vi "Auto_PID_Drive.vi"(0 "Power":dbl, 1 "dt (s)":dbl=10.0 format="%.3f", 5 "Turning":dbl, 7 "PID Gains":T1={"P"=0.09, "I"=0.9, "D"=0.001, "F"=0.0, "IZone"=0.0}, 9 "Yaw":dbl=-13.119872265000097, 11 "Turning_Setpoint":dbl, 12 "Turning_PID_Enable":bool) -> (4 "Power":dbl, 6 "Turning":dbl)   [LabVIEW 2019, in "ArgosLib.lvlib"]
uses:
  ArgosLib.lvlib
  Config/ConfigComponents/TypeDefs/Config_PIDParams.ctl
  <vilib>/addons/control/pid/pid.llb/PID (DBL).vi
  <vilib>/Rock Robotics/Network Tables/NT Write Number.vi
  <vilib>/addons/control/pid/NI_PID_pid.lvlib
  <vilib>/Rock Robotics/Network Tables/NT Read Number.vi
panel:
  out "Error":dbl
  out "Waveform Chart 2":dbl(graph)
  out "Waveform Chart":cluster{"Turning_Setpoint":dbl, "Yaw":dbl}(graph)={"Turning_Setpoint"=0.0, "Yaw"=-13.119872265000097}
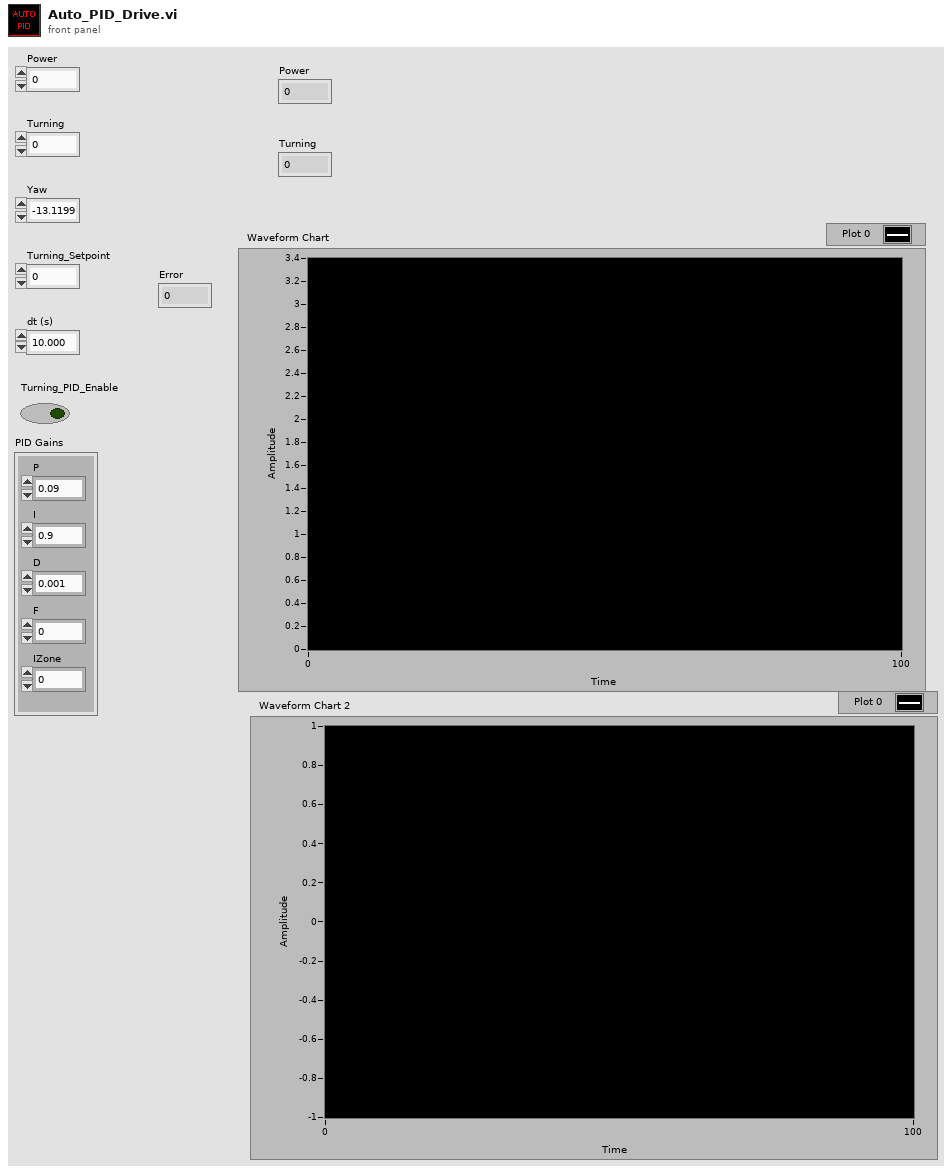
[diagram p1: front panel]
types:
  T1 = typedef "ArgosLib.lvlib/Config_PIDParams.ctl" = cluster{"P":dbl, "I":dbl, "D":dbl, "F":dbl, "IZone":dbl}
  T2 = cluster{"Power":dbl, "Yaw":dbl, "Turning_PID_Enable":bool, "Turning":dbl, "Turning_Setpoint":dbl, "PID Gains":T1, "dt (s)":dbl}
  T3 = cluster{"proportional gain (Kc)":dbl, "integral time (Ti, min)":dbl, "derivative time (Td, min)":dbl}
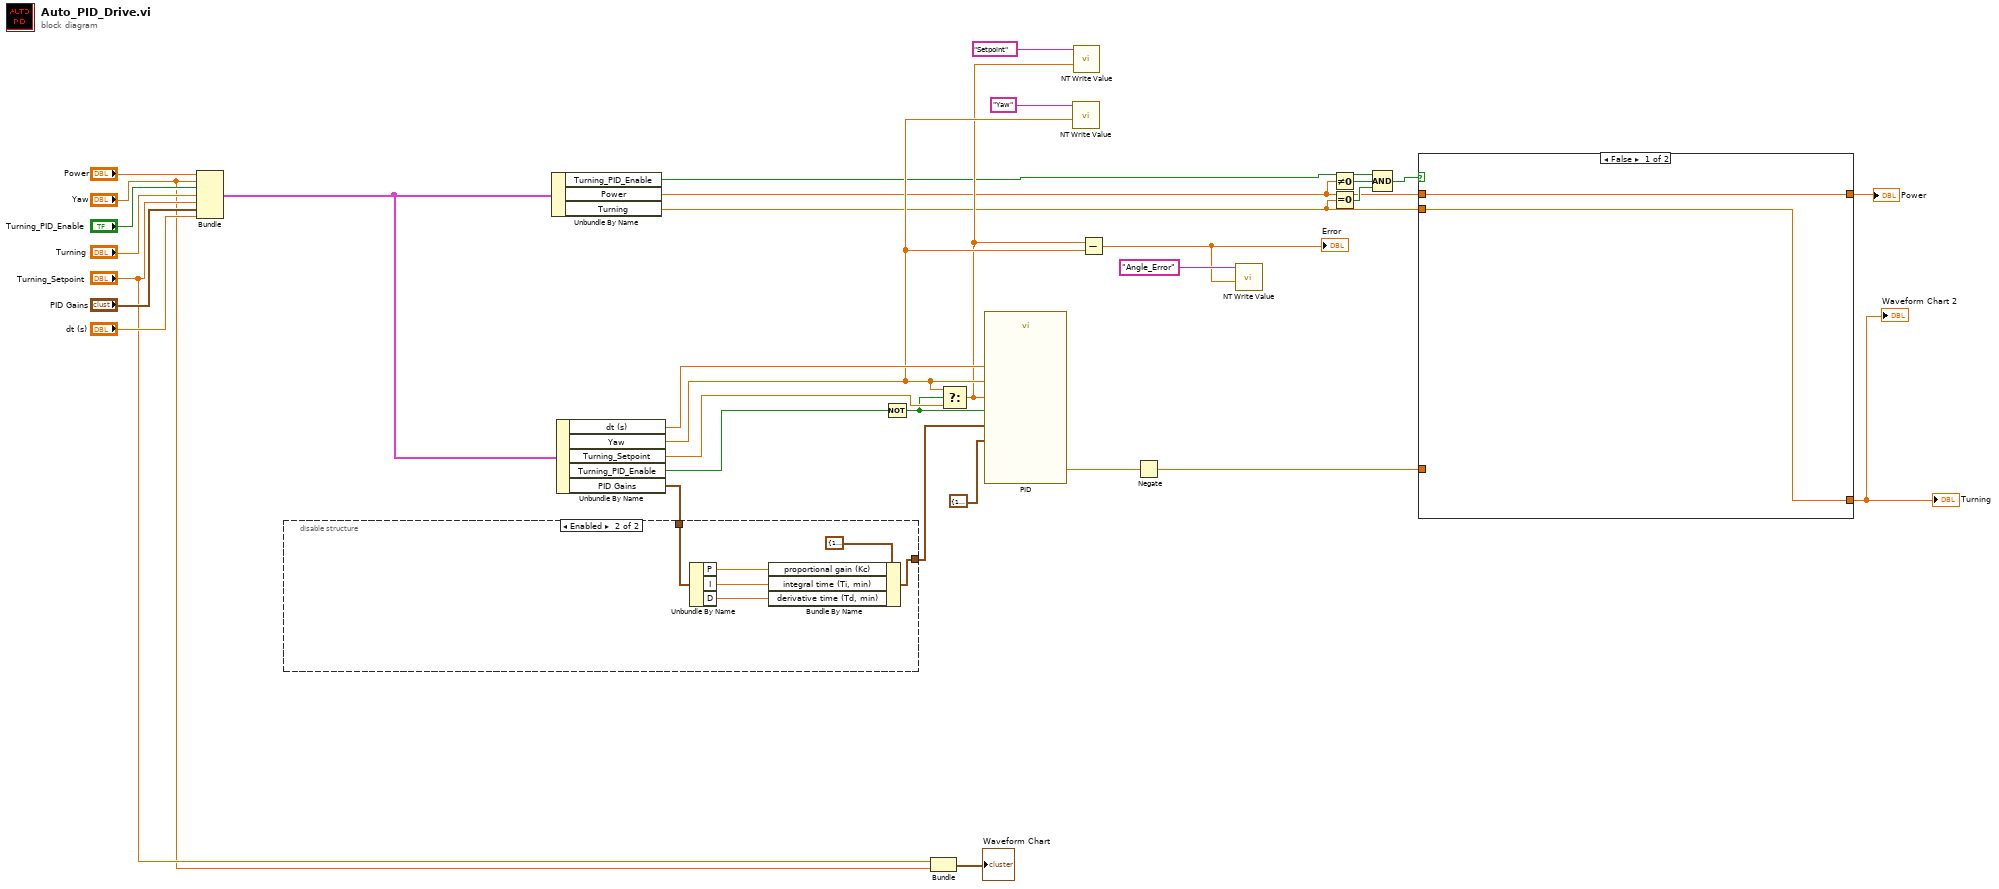
[diagram p0: block diagram]
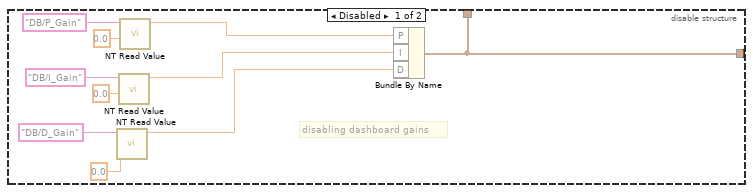
[diagram p2: hidden frame]
diagram:
  n1 = Bundle("Power"="Power", "Yaw"="Yaw", "Turning_PID_Enable"="Turning_PID_Enable", "Turning"="Turning", "Turning_Setpoint"="Turning_Setpoint", "PID Gains"="PID Gains", "dt (s)"="dt (s)") -> (w23:T2)  [unwired: 1 in]
  n2 = Unbundle By Name(w23) -> ("Turning_PID_Enable"=w7:bool, "Power"=w1:dbl, "Turning"=w6:dbl)
  n3 = Unbundle By Name(w23) -> ("dt (s)"=w20:dbl, "Yaw"=w12:dbl, "Turning_Setpoint"=w18:dbl, "Turning_PID_Enable"=w19:bool, "PID Gains"=w9:T1)
  n4 = disable-structure shown="Enabled" {
    disable-tunnel: [w42 w44] -> w8
    disable-tunnel: [w33 _] -> _
    disable-tunnel: w9 -> [w33 w49]
    frame Disabled {
      # "disabling dashboard gains"
      n5 = call-poly <vilib>:"NT Read Value.vi"("Default Value"=0.0, "Name"="DB/D_Gain" ("refnum name")) -> ("Numeric"=w35:dbl)  [unwired: 8 in, 1 out]
      n6 = call-poly <vilib>:"NT Read Value.vi"("Default Value"=0.0, "Name"="DB/I_Gain" ("refnum name")) -> ("Numeric"=w36:dbl)  [unwired: 8 in, 1 out]
      n7 = call-poly <vilib>:"NT Read Value.vi"("Default Value"=0.0, "Name"="DB/P_Gain" ("refnum name")) -> ("Numeric"=w37:dbl)  [unwired: 8 in, 1 out]
      n8 = Bundle By Name(cluster=w33, "P"=w37, "I"=w36, "D"=w35) -> (w42:T1)
    }
    frame Enabled {
      n9 = Unbundle By Name(w49) -> ("P"=w47:dbl, "I"=w46:dbl, "D"=w45:dbl)
      n10 = Bundle By Name(cluster=T3 {"proportional gain (Kc)"=1.0, "integral time (Ti, min)"=0.01, "derivative time (Td, min)"=0.0} ("PID gains"), "proportional gain (Kc)"=w47, "integral time (Ti, min)"=w46, "derivative time (Td, min)"=w45) -> (w44:T3)
    }
  }
  n11 = Not(x=w19) -> (.not. x?=w17:bool)
  n12 = Bundle("Turning_Setpoint"="Turning_Setpoint", "Yaw"="Yaw") -> (→"Waveform Chart":cluster{"Turning_Setpoint":dbl, "Yaw":dbl})  [unwired: 1 in]
  n13 = Select(t=w12, s=w17, f=w18) -> (s? t:f=w11:dbl)
  n14 = call-poly <vilib>:"PID.vi"("reinitialize? (F)"=w17, "output range"=cluster{"output high":dbl, "output low":dbl} {"output high"=1.0, "output low"=-1.0}, "dt (s)"=w20, "PID gains"=w8, "process variable"=w12, "setpoint"=w11) -> ("output"=w10:dbl)  [unwired: 4 in, 1 out]
  n15 = call-poly <vilib>:"NT Write Value.vi"("Numeric"=w12, "Name"="Yaw") -> ()  [unwired: 9 in, 1 out]
  n16 = call-poly <vilib>:"NT Write Value.vi"("Numeric"=w11, "Name"="Setpoint") -> ()  [unwired: 9 in, 1 out]
  n17 = Subtract(x=w11, y=w12) -> (x-y=w15:dbl)
  "Error" <- w15
  n18 = Negate(x=w10) -> (-x=w4:dbl)
  n19 = call-poly <vilib>:"NT Write Value.vi"("Numeric"=w15, "Name"="Angle_Error") -> ()  [unwired: 9 in, 1 out]
  n20 = Not Equal To 0?(x=w1) -> (x != 0?=w3:bool)
  n21 = Equal To 0?(x=w6) -> (x = 0?=w2:bool)
  n22 = Compound Arithmetic op=AND(w7, w3, w2) -> (w5:bool)
  n23 = case shown="False" w5 {
    tunnel: w1 -> [w51 w53]
    tunnel: w6 -> [w50 _]
    tunnel: [w51 w53] -> w28
    tunnel: [w50 w52] -> w22
    tunnel: w4 -> [_ w52]
    frame False {
    }
    frame True {
    }
  }
  "Power" <- w28
  "Turning" <- w22
  "Waveform Chart 2" <- w22
